vi "Test Empty Hardware Buffer.vi"() -> (0 "error out":errorcluster)   [LabVIEW 2026]
doc: "BUF-002: a valid empty queue returns error 5100, not success or an unlimited wait."
uses:
  source/framework/Hardware/Hardware.lvclass
  source/framework/Hardware/Hardware.lvclass/Hardware.ctl
  <vilib>/addons/_JKI Toolkits/Caraya/classes/Test/Test.lvclass
  <vilib>/addons/_JKI Toolkits/Caraya/classes/Assert/Assert.lvclass
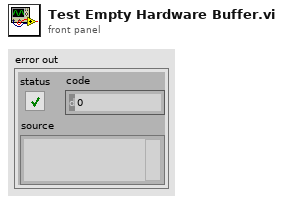
[diagram p1: front panel]
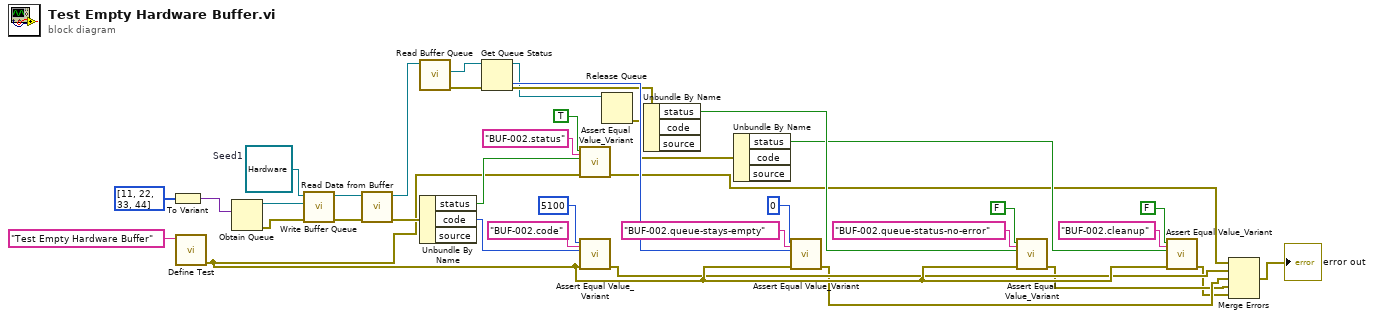
[diagram p0: block diagram]
diagram:
  w33 = refnum<class "Hardware.lvclass"> refnum  # Seed1
  n1 = To Variant(anything=i32[] [11, 22, 33, 44]) -> (Variant=w35:variant)
  n2 = call <vilib>:"Define Test.vi"("Label (VI Title)"="Test Empty Hardware Buffer") -> ("error out"=w9:errorcluster)  [unwired: 9 in, 1 out]
  n3 = Obtain Queue(element data type=w35) -> (queue out=w32:refnum<queue>, error out=w34:errorcluster)  [unwired: 4 in, 1 out]
  n4 = call "Write Buffer Queue.vi"("error in (no error)"=w34, "Buffer Queue"=w32, "Hardware in"=w33) -> ("error out"=w31:errorcluster, "Hardware out"=w30:refnum<class "Hardware.lvclass">)  [unwired: 7 in]
  n5 = call "Read Data from Buffer.vi"("error in (no error)"=w31, "Hardware in"=w30) -> ("error out"=w29:errorcluster, "Hardware out"=w22:refnum<class "Hardware.lvclass">)  [unwired: 7 in, 1 out]
  n6 = call "Read Buffer Queue.vi"("Hardware in"=w22) -> ("error out"=w21:errorcluster, "Buffer Queue"=w20:refnum<queue>)  [unwired: 8 in, 1 out]
  n7 = Unbundle By Name(w29) -> ("status"=w28:bool, "code"=w25:i32)  [unwired: 1 out]
  n8 = Get Queue Status(queue=w20, error in (no error)=w21) -> (queue out=w12:refnum<queue>, error out=w16:errorcluster, # elements in queue=w19:i32)  [unwired: 1 in, 5 out]
  n9 = call <vilib>:"Assert Equal Value_Variant.vi"("Label"="BUF-002.status", "error in (no error)"=w9, "Actual"=w28, "Expected"=TRUE) -> ("error out"=w6:errorcluster)  [unwired: 6 in, 1 out]
  n10 = call <vilib>:"Assert Equal Value_Variant.vi"("Label"="BUF-002.code", "error in (no error)"=w9, "Actual"=w25, "Expected"=5100) -> ("error out"=w5:errorcluster)  [unwired: 6 in, 1 out]
  n11 = Release Queue(queue=w12) -> (error out=w11:errorcluster)  [unwired: 2 in, 2 out]
  n12 = Unbundle By Name(w16) -> ("status"=w15:bool)  [unwired: 2 out]
  n13 = Unbundle By Name(w11) -> ("status"=w10:bool)  [unwired: 2 out]
  n14 = call <vilib>:"Assert Equal Value_Variant.vi"("Label"="BUF-002.queue-stays-empty", "error in (no error)"=w9, "Actual"=w19, "Expected"=0) -> ("error out"=w4:errorcluster)  [unwired: 6 in, 1 out]
  n15 = call <vilib>:"Assert Equal Value_Variant.vi"("Label"="BUF-002.queue-status-no-error", "error in (no error)"=w9, "Actual"=w15, "Expected"=FALSE) -> ("error out"=w3:errorcluster)  [unwired: 6 in, 1 out]
  n16 = call <vilib>:"Assert Equal Value_Variant.vi"("Label"="BUF-002.cleanup", "error in (no error)"=w9, "Actual"=w10, "Expected"=FALSE) -> ("error out"=w2:errorcluster)  [unwired: 6 in, 1 out]
  n17 = Merge Errors(w6, w5, w4, w3, w2) -> (→"error out":errorcluster)
